vi "VIH Utility - FILE - Find Valid Root Directory of a Path.vi"(8 "error in":errorcluster, 11 "Path in":path) -> (0 "error out":errorcluster, 2 "relative path from Root directory":path, 3 "Root directory path":path)   [LabVIEW 2014]
doc: "::: VI Helpeks :::\nCopyright (c) 2000-2026 Konstantin Shifershteyn. All rights reserved."
panel:
  # "VI Helpeks\nCopyright (c) 2012-2026 Konstantin Shifershteyn"
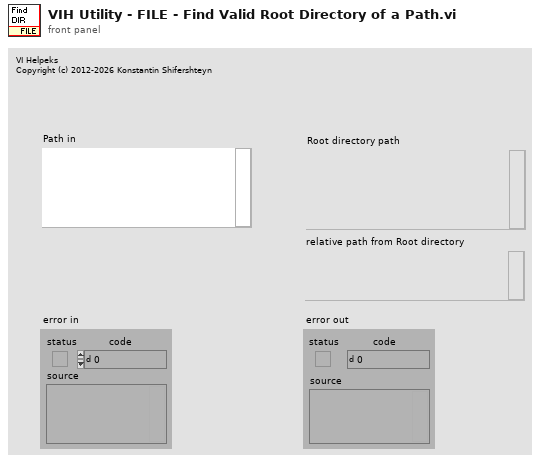
[diagram p1: front panel]
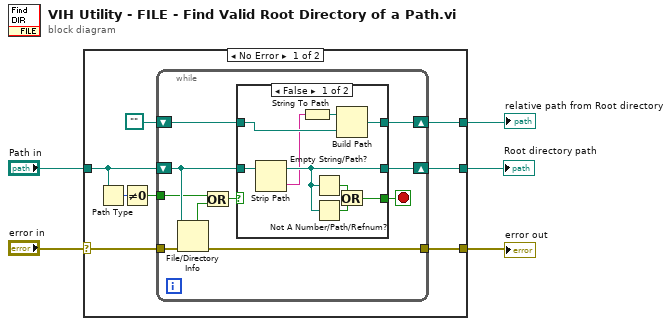
[diagram p0: block diagram]
diagram:
  n1 = case shown="No Error" "error in" {
    selector: "error in" -> [w9 w36]
    tunnel: [w13 w37] -> w3
    tunnel: [w8 w36] -> w5
    tunnel: "Path in" -> [w12 w37]
    tunnel: [w6 _] -> w2
    frame No Error {
      n2 = Path Type(1:w12) -> (0:w11:i16)
      n3 = Not Equal To 0?(x=w11) -> (x != 0?=w10:bool)
      n4 = while {
        shift-right: [w22] -> w13
        shift-left: w12 -> [w23]
        tunnel: [w16] -> w8
        tunnel: w9 -> [w21]
        tunnel: w10 -> [w17]
        shift-right: [w14] -> w6
        shift-left: path "" -> [w15]
        stop <- w20 stop-if-true
        n5 = File/Directory Info(path=w23, error in=w21) -> (directory=w19:bool, error out=w16:errorcluster)  [unwired: 5 out]
        n6 = Or(x=w17, y=w19) -> (x .or. y?=w18:bool)
        n7 = case shown="False" w18 {
          selector: w18 -> [_ w35]
          tunnel: [w28 w35] -> w20
          tunnel: w23 -> [w32 w34]
          tunnel: [w31 w34] -> w22
          tunnel: w15 -> [w26 w33]
          tunnel: [w27 w33] -> w14
          frame False {
            n8 = Strip Path(path=w32) -> (stripped path=w31:path, name=w25:string)
            n9 = String To Path(string=w25) -> (path=w24:path)
            n10 = Empty String/Path?(string/path=w31) -> (empty?=w30:bool)
            n11 = Not A Number/Path/Refnum?(number/path/refnum=w31) -> (NaN/Path/Refnum?=w29:bool)
            n12 = Build Path(base path=w24, name or relative path=w26) -> (appended path=w27:path)
            n13 = Or(x=w30, y=w29) -> (x .or. y?=w28:bool)
          }
          frame True {
          }
        }
      }
    }
    frame Error {
    }
  }
  "Root directory path" <- w3
  "error out" <- w5
  "relative path from Root directory" <- w2
